vi "Test_C_Smoke.vi"() -> ()   [LabVIEW 2021]
uses:
  CANsub_C.lvlib
  C_Info.ctl
  common/Typedefs/Bit_Timing.ctl
  common/CANsub_Common.lvlib
panel:
  out "error out":errorcluster
  out "data sample point out":dbl
  out "nominal sample point out":dbl
  out "Bit_Timing":T1
  out "crc32":u32 format="%.0x"
  out "C_Info":T2
  # "Expected for Version 1.3"
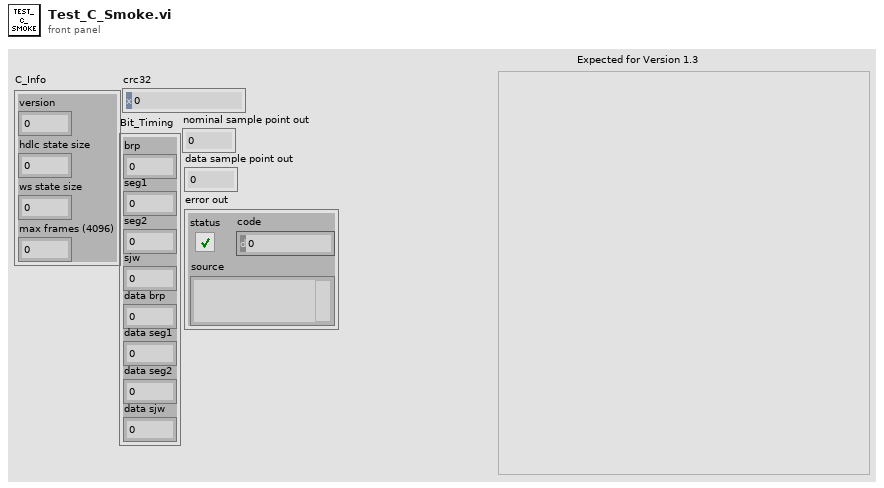
[diagram p1: front panel]
types:
  T1 = typedef "CANsub_Common.lvlib/Bit_Timing.ctl" = cluster{"brp":u16, "seg1":u16, "seg2":u16, "sjw":u16, "data brp":u16, "data seg1":u16, "data seg2":u16, "data sjw":u16}
  T2 = typedef "CANsub_C.lvlib/C_Info.ctl" = cluster{"version":u32, "hdlc state size":i32, "ws state size":i32, "max frames (4096)":i32}
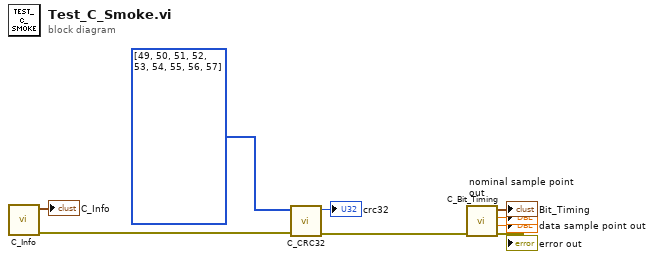
[diagram p0: block diagram]
diagram:
  n1 = call "C_Info.vi"() -> ("error out"=w8:errorcluster, "C_Info"=→"C_Info":T2)  [unwired: 10 in]
  n2 = call "C_CRC32.vi"("error in (no error)"=w8, "data"=u8[] [49, 50, 51, 52, 53, 54, 55, 56, 57]) -> ("error out"=w5:errorcluster, "crc32"=→"crc32":u32)  [unwired: 8 in]
  n3 = call "C_Bit_Timing.vi"("error in (no error)"=w5) -> ("error out"=→"error out":errorcluster, "data sample point out"=→"data sample point out":dbl, "nominal sample point out"=→"nominal sample point out":dbl, "Bit_Timing"=→"Bit_Timing":T1)  [unwired: 7 in]
